vi "getExceptionMessage.vi"(9 "exception":i32, 11 "Job in":refnum<class "Job.lvclass">) -> (0 "exception message":string, 1 "exception dup":i32, 3 "warning?":bool)   [LabVIEW 2013, in "openCronJob.lvlib" / "Job.lvclass"]
uses:
  Job.lvclass
  <vilib>/Utility/error.llb/DialogType.ctl
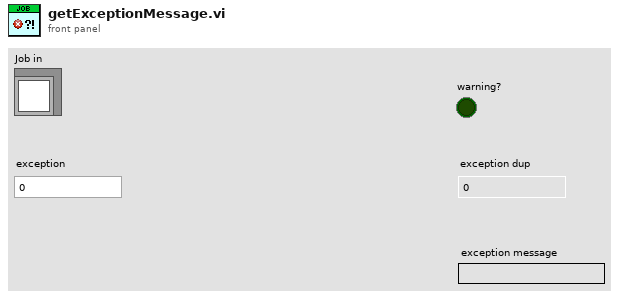
[diagram p1: front panel]
types:
  T1 = typedef "DialogType.ctl" = u16
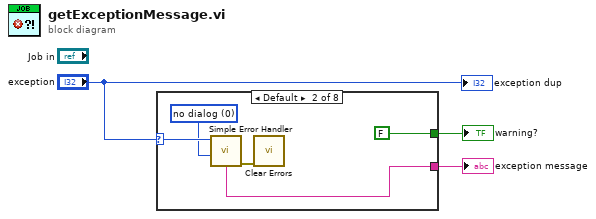
[diagram p0: block diagram]
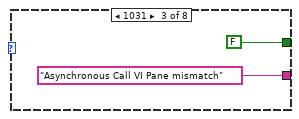
[diagram p3: hidden frame]
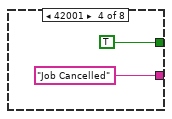
[diagram p4: hidden frame]
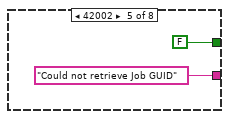
[diagram p5: hidden frame]
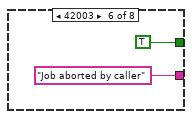
[diagram p6: hidden frame]
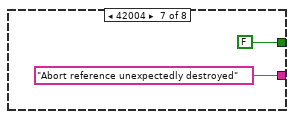
[diagram p7: hidden frame]
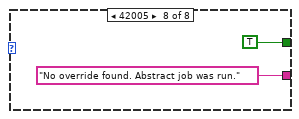
[diagram p8: hidden frame]
diagram:
  n1 = case shown="Default" "exception" {
    selector: "exception" -> [_ w7 _ _ _ _ _ _]
    tunnel: [_ w5 "Asynchronous Call VI Pane mismatch" ("error message") "Job Cancelled" ("error message") "Could not retrieve Job GUID" ("error message") "Job aborted by caller" ("error message") "Abort reference unexpectedly destroyed" ("error message") "No override found. Abstract job was run." ("error message")] -> w3
    tunnel: [_ FALSE FALSE TRUE FALSE TRUE FALSE TRUE] -> w1
    frame 0 {
    }
    frame Default {
      w6 = T1 0 items=["no dialog", "OK message", "continue or stop message", "OK message + warnings", "continue/stop + warnings"] ("type of dialog (OK msg:1)")
      n2 = call <vilib>:"Simple Error Handler.vi"("error code (no error:0)"=w7, "type of dialog (OK msg:1)"=w6) -> ("error out"=w4:errorcluster, "message"=w5:string)  [unwired: 3 in, 3 out]
      n3 = call <vilib>:"Clear Errors.vi"("error in (no error)"=w4) -> ()  [unwired: 6 in, 1 out]
    }
    frame 1031 {
    }
    frame 42001 {
    }
    frame 42002 {
    }
    frame 42003 {
    }
    frame 42004 {
    }
    frame 42005 {
    }
  }
  "exception message" <- w3
  "warning?" <- w1
  "exception dup" <- "exception"
